vi "libssh2_userauth_banner.vi"(8 "error in (no error)":errorcluster, 11 "session":T1) -> (0 "error out":errorcluster, 2 "banner":string)   [LabVIEW 2017, in "libssh2.lvlib"]
doc: "Get the banner that was sent by the server during user authentication."
uses:
  libssh2.lvlib
  Session Refnum.ctl
  Not A Session.vi
  <vilib>/Utility/error.llb/Error Cluster From Error Code.vi
  Global Settings.vi
  Read Session Refnum.vi
  <vilib>/Utility/semaphor.llb/Acquire Semaphore.vi
  <vilib>/Utility/semaphor.llb/Release Semaphore.vi
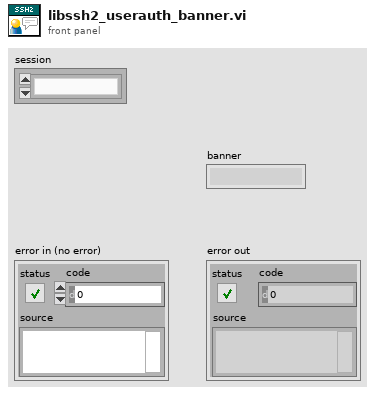
[diagram p1: front panel]
types:
  T1 = typedef "libssh2.lvlib/Session Refnum.ctl" = refnum<k1>
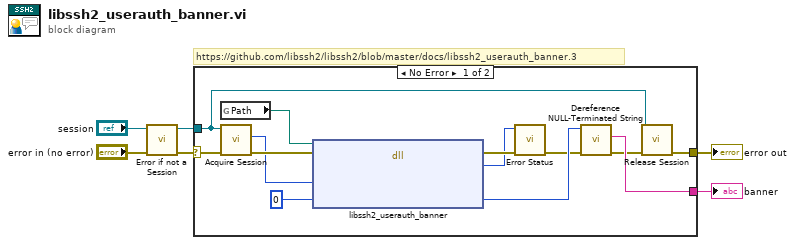
[diagram p0: block diagram]
diagram:
  # "https://github.com/libssh2/libssh2/blob/master/docs/libssh2_userauth_banner.3"
  n1 = call "Error if not a Session.vi"("error in (no error)"="error in (no error)", "session"="session") -> ("error out"=w3:errorcluster, "session out"=w1:T1)  [unwired: 8 in]
  n2 = case shown="No Error" w3 {
    selector: w3 -> [w15 w20]
    tunnel: [w8 w20] -> w6
    tunnel: [w18 _] -> w5
    tunnel: w1 -> [w7 _]
    frame No Error {
      n3 = global read "Global Settings.vi" "Path"() -> (w11:path)
      n4 = call "Acquire Session.vi"("error in (no error)"=w15, "session"=w7) -> ("error out"=w17:errorcluster, "LIBSSH2_SESSION*"=w16:u64)  [unwired: 7 in, 1 out]
      n5 = dll-call lib="?" fn="libssh2_userauth_banner"(path in=w11, error in=w17, "session"=w16, "banner"=u64 0) -> (error out=w13:errorcluster, "return value"=w9:i32, "banner"=w14:u64)  [unwired: 2 in, 1 out]
      n6 = call "Error Status.vi"("error in (no error)"=w13, "return value"=w9) -> ("error out"=w10:errorcluster)  [unwired: 8 in, 1 out]
      n7 = call "Dereference NULL-Terminated String.vi"("error in (no error)"=w10, "char*"=w14) -> ("error out"=w12:errorcluster, "string"=w18:string)  [unwired: 8 in]
      n8 = call "Release Session.vi"("error in (no error)"=w12, "session"=w7) -> ("error out"=w8:errorcluster)  [unwired: 9 in]
    }
    frame Error {
    }
  }
  "error out" <- w6
  "banner" <- w5
